vi "Game_Undo.vi"(0 "Board State":T1={"Grid"=array15x15[225 elements], "Move History"=[], "Last Move"={"Row"=-1, "Col"=-1, "Stone"=enum."Empty"}}, 5 "Count":i32=2, 11 "error in":errorcluster) -> (4 "Board State out":T1={"Grid"=array15x15[225 elements], "Move History"=[], "Last Move"={"Row"=-1, "Col"=-1, "Stone"=enum."Empty"}}, 6 "Undone":i32, 15 "error out":errorcluster)   [LabVIEW 2026]
doc: "무르기: Move History 끝에서 Count개를 지우고 Grid 칸을 비운다(기본 2 = 플레이어+AI 한 수씩).\nUndone = 실제로 되돌린 수."
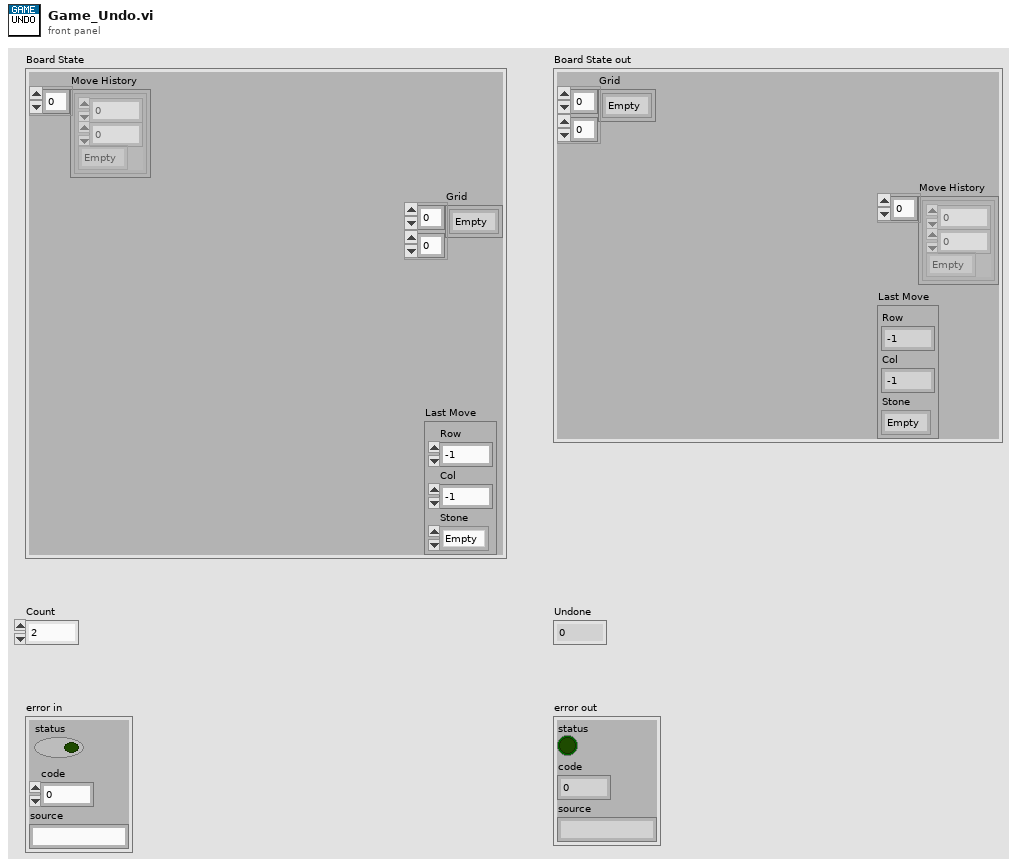
[diagram p1: front panel]
types:
  T1 = cluster{"Grid":enum8{"Empty", "Black", "White"}[][], "Move History":cluster{"Row":i32, "Col":i32, "Stone":enum8{"Empty", "Black", "White"}}[], "Last Move":cluster{"Row":i32, "Col":i32, "Stone":enum8{"Empty", "Black", "White"}}}
  T2 = cluster{"Row":i32, "Col":i32, "Stone":enum8{"Empty", "Black", "White"}}
  T3 = cluster{"Row":i32, "Col":i32, "Stone":enum8{"Empty", "Black", "White"}}[]
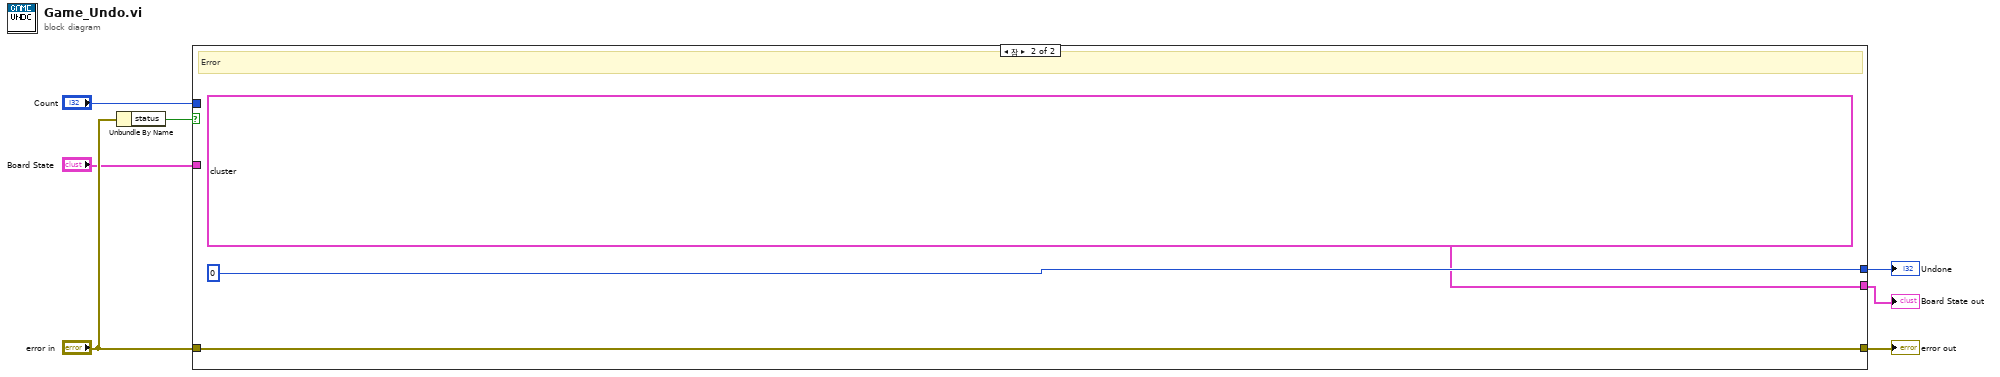
[diagram p0: block diagram]
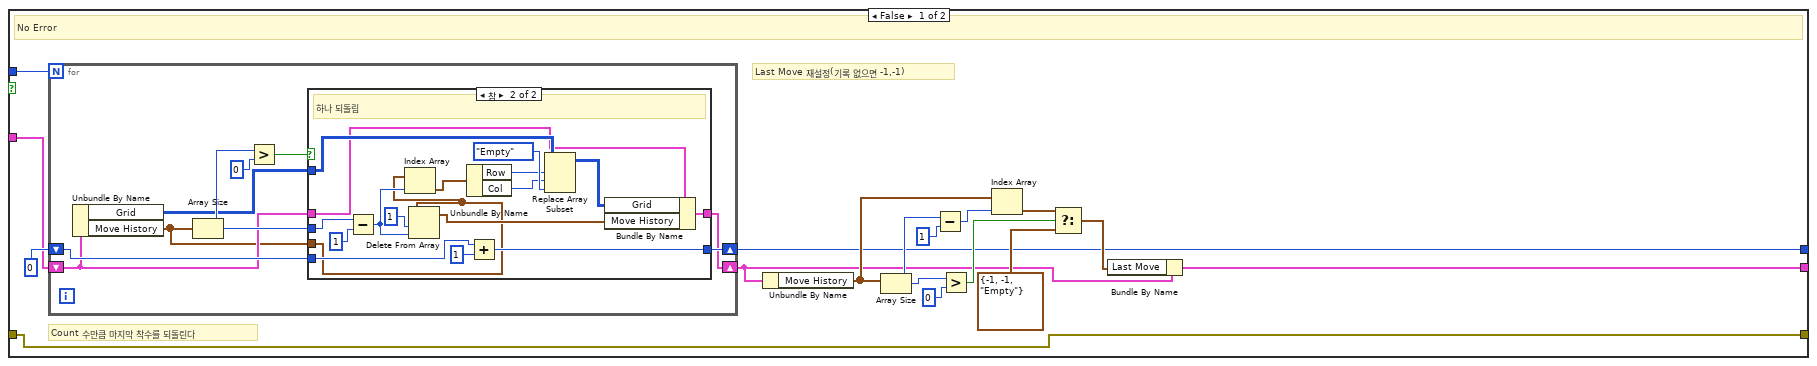
[diagram p2: hidden frame]
diagram:
  n1 = Unbundle By Name("error in") -> ("status"=w4:bool)
  n2 = case shown="참" w4 {
    tunnel: "Board State" -> [w8 _]
    tunnel: "Count" -> [w9 _]
    tunnel: "error in" -> [w10 w52]
    tunnel: [w13 0] -> w6
    tunnel: [w10 w52] -> w7
    tunnel: [w23 T1 {"Grid"=array15x15[225 elements], "Move History"=[], "Last Move"={"Row"=-1, "Col"=-1, "Stone"=enum."Empty"}}] -> w5
    frame False {
      # "Last Move 재설정(기록 없으면 -1,-1)"
      # "Count 수만큼 마지막 착수를 되돌린다"
      # "No Error"
      n3 = for {
        N: w9 -> [_]
        shift-right: [w32] -> w13
        shift-left: 0 -> [w30]
        shift-right: [w31] -> w12
        shift-left: w8 -> [w26]
        n4 = Unbundle By Name(w26) -> ("Grid"=w24:enum8{"Empty", "Black", "White"}[][], "Move History"=w25:T3)
        n5 = Array Size(array=w25) -> (size(s)=w27:i32)
        n6 = Greater?(x=w27, y=0) -> (0:w29:bool)
        n7 = case shown="참" w29 {
          tunnel: w30 -> [w34 w39]
          tunnel: w26 -> [w33 w35]
          tunnel: w24 -> [_ w36]
          tunnel: w25 -> [_ w37]
          tunnel: [w34 w51] -> w32
          tunnel: w27 -> [_ w38]
          tunnel: [w33 w49] -> w31
          frame False {
            # "기록 없음"
          }
          frame True {
            # "하나 되돌림"
            n8 = Subtract(x=w38, y=1) -> (x-y=w41:i32)
            n9 = Index Array(array=w37, index=w41) -> (element=w42:T2)
            n10 = Delete From Array(array=w37, length=1, index=w41) -> (array with subset deleted=w48:T3)  [unwired: 1 out]
            n11 = Unbundle By Name(w42) -> ("Row"=w43:i32, "Col"=w44:i32)
            n12 = Add(x=w39, y=1) -> (x+y=w51:i32)
            n13 = Replace Array Subset(array=w36, new element=enum8{"Empty", "Black", "White"}."Empty", index (row)=w43, index (col)=w44) -> (w46:enum8{"Empty", "Black", "White"}[][])
            n14 = Bundle By Name(cluster=w35, "Grid"=w46, "Move History"=w48) -> (w49:T1)
          }
        }
      }
      n15 = Unbundle By Name(w12) -> ("Move History"=w14:T3)
      n16 = Array Size(array=w14) -> (size(s)=w15:i32)
      n17 = Subtract(x=w15, y=1) -> (x-y=w19:i32)
      n18 = Greater?(x=w15, y=0) -> (0:w17:bool)
      n19 = Index Array(array=w14, index=w19) -> (element=w20:T2)
      n20 = Select(t=w20, s=w17, f=T2 {"Row"=-1, "Col"=-1, "Stone"=enum."Empty"}) -> (s? t:f=w22:T2)
      n21 = Bundle By Name(cluster=w12, "Last Move"=w22) -> (w23:T1)
    }
    frame True {
      # "Error"
    }
  }
  "Board State out" <- w5
  "Undone" <- w6
  "error out" <- w7
